vi "VM - Variable Info.vi"(7 "VC Handle":T1=-1, 8 "error in":errorcluster, 11 "name_spec":string) -> (0 "error out":errorcluster, 1 "var type":u32, 2 "alias":string, 3 "var name":string, 4 "has history":bool, 5 "var VC Handle":T1=-1)   [LabVIEW 2021]
doc: "This VI returns information about a variable. Refer to the VI help for more details.\n\n<b>VC Handle</b> specifies the handle of the variable context. To get information on a global variable, pass the value of -1 to this input. This input is ignored if the <b>name_spec</b> control refers to a variable by an alias. \n\n<b>name_spec</b> is the name specifier of the desired variable. Usually, it is merely a variable name; however, its generic format is '[name][=alias]', where either 'name' or '=alias' can be omitted but not both.\n\n<b>var VC Handle</b> indicator returns the handle of the context where the specified variable resides. It can differ from <b>VC Handle</b> if <b>name_spec</b> refers to a variable by an alias.\n\n<b>alias</b> indicator returns the alias associated with the specified variable.\n\n<b>var type</b> indicator returns the data type code of the variable.\n\n<b>has history</b> indicator returns TRUE if the variable has a history attached.\n\n::: CalcExpress Toolkit :::\nCopyright (c) 2000-2026 Konstantin Shifershteyn. All rights reserved."
uses:
  cetypes.llb/VarMan Variable Context Handle.ctl
  cetypes.llb/VarMan Error Code.ctl
  cersrc/celveng32.dll
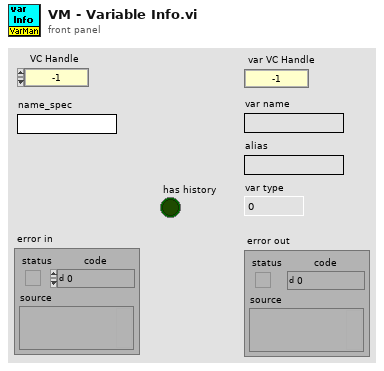
[diagram p1: front panel]
types:
  T1 = typedef "VarMan Variable Context Handle.ctl" = i32
  T2 = typedef "VarMan Error Code.ctl" = u16
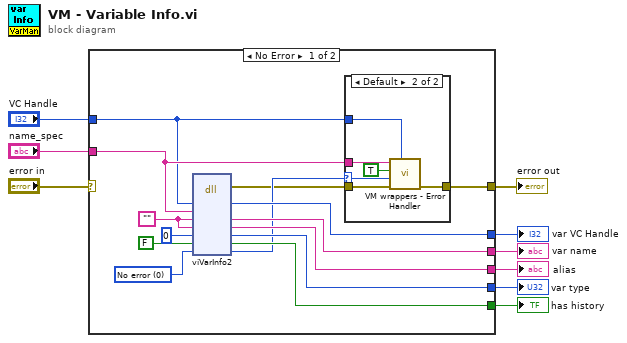
[diagram p0: block diagram]
diagram:
  n1 = case shown="No Error" "error in" {
    selector: "error in" -> [_ w32]
    tunnel: [w23 w32] -> w9
    tunnel: [w22 _] -> w8
    tunnel: "name_spec" -> [w20 _]
    tunnel: "VC Handle" -> [w19 w31]
    tunnel: [w18 _] -> w5
    tunnel: [w17 _] -> w4
    tunnel: [w16 _] -> w3
    tunnel: [w15 w31] -> w2
    frame No Error {
      w12 = T2 0 items=["No error", "Invalid variable type", "Variable not found", "Variable already exists", "Invalid context handle", "Input error", "Invalid data format", "No history attached", "History already attached", "Invalid history parameters", "Wrong variable name", "Wrong alias name", "Non-unique alias", "Alias not found", "No alias associated", "Alias already associated", "Wrong context name", "Non-unique context name", "Context name not found", "Invalid parameter", "Generic error", "Memory Full", "Unrecognized LV error", "Unknown error code"] ("VarMan error")
      w13 = "" ("Empty String Constant")
      n2 = dll-call lib="C:/LV Projects/CalcExpress 40 LV2021/vi.lib/addons/CalcExpress/cersrc/celveng*.dll" fn="viVarInfo2"("vch"=w19, "nspec"=w20, "name"=w13, "alias"=w13, "type"=u32 0, "fHist"=FALSE, "errc"=w12) -> (error out=w10:errorcluster, "vch"=w15:i32, "name"=w16:string, "alias"=w17:string, "type"=w18:u32, "fHist"=w22:bool, "errc"=w11:T2)  [unwired: 5 in, 1 out]
      n3 = case shown="Default" w11 {
        selector: w11 -> [_ w25]
        tunnel: w10 -> [w24 w30]
        tunnel: w19 -> [_ w29]
        tunnel: [w24 w28] -> w23
        tunnel: w20 -> [_ w26]
        frame 0 {
        }
        frame Default {
          n4 = call "VM wrappers - Error Handler.vi"("VC Handle"=w29, "error before"=w30, "VarMan error"=w25, "show name spec (F)"=TRUE, "name spec"=w26) -> ("error out"=w28:errorcluster)  [unwired: 5 in, 1 out]
        }
      }
    }
    frame Error {
    }
  }
  "error out" <- w9
  "var VC Handle" <- w2
  "var name" <- w3
  "alias" <- w4
  "var type" <- w5
  "has history" <- w8
